vi "测试ezcad.vi"() -> ()   [LabVIEW 2017]
uses:
  C:/Users/skate/OneDrive/0_Github_App_/lazer_cad/lazer_cad_demo/LazerClassLibrary/bin/x86/Debug/LazerClassLibrary.dll
  LazerClassLibrary/bin/x86/Debug/LazerClassLibrary.dll
panel:
  out "Mark":i32
  out "WaitForMarkCompleted":i32
  in  "替换名称":string="TA"
  in  "替换内容":string="123456"
  in  "模板目录":path
  in  "程序目录":path
  out "Close":i32
  out "LoadEzdFile":i32
  out "Initialize":i32
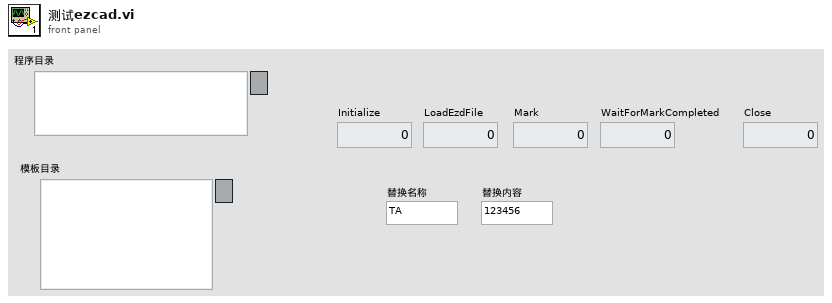
[diagram p1: front panel]
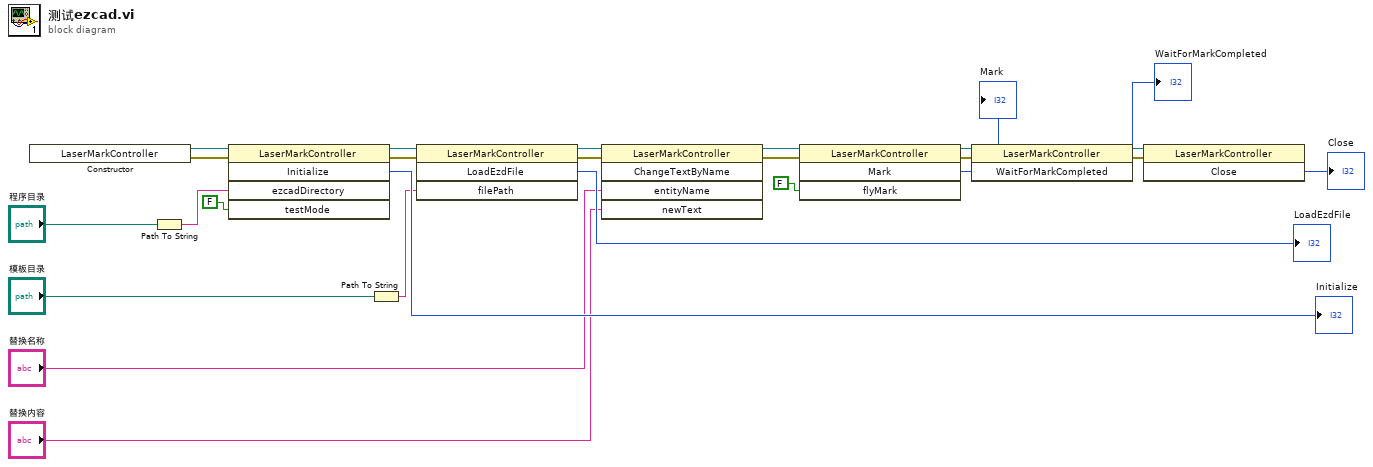
[diagram p0: block diagram]
diagram:
  n1 = constructor class="LaserMarkController"() -> (reference out=w25:refnum<k24>, error out=w24:errorcluster)  [unwired: 3 in, 1 out]
  n2 = Path To String(path="程序目录") -> (string=w14:string)
  n3 = invoke on="调用节点" class="LaserMarkController" method="Initialize"(reference=w25, error in=w24, "ezcadDirectory"=w14, "testMode"=FALSE) -> (reference out=w23:refnum<k24>, error out=w22:errorcluster, "Initialize"=→"Initialize":i32)  [unwired: 1 in, 2 out]
  n4 = Path To String(path="模板目录") -> (string=w16:string)
  n5 = invoke on="调用节点" class="LaserMarkController" method="LoadEzdFile"(reference=w23, error in=w22, "filePath"=w16) -> (reference out=w13:refnum<k24>, error out=w12:errorcluster, "LoadEzdFile"=→"LoadEzdFile":i32)  [unwired: 1 in, 1 out]
  n6 = invoke on="调用节点" class="LaserMarkController" method="ChangeTextByName"(reference=w13, error in=w12, "entityName"="替换名称", "newText"="替换内容") -> (reference out=w9:refnum<k24>, error out=w7:errorcluster)  [unwired: 1 in, 3 out]
  n7 = invoke on="调用节点" class="LaserMarkController" method="Mark"(reference=w9, error in=w7, "flyMark"=FALSE) -> (reference out=w5:refnum<k24>, error out=w6:errorcluster, "Mark"=→"Mark":i32)  [unwired: 1 in, 1 out]
  n8 = invoke on="调用节点" class="LaserMarkController" method="WaitForMarkCompleted"(reference=w5, error in=w6) -> (reference out=w4:refnum<k24>, error out=w3:errorcluster, "WaitForMarkCompleted"=→"WaitForMarkCompleted":i32)  [unwired: 1 in]
  n9 = invoke on="调用节点" class="LaserMarkController" method="Close"(reference=w4, error in=w3) -> ("Close"=→"Close":i32)  [unwired: 1 in, 2 out]
